vi "Ch_Defaults.vi"(11 "error in":errorcluster) -> (4 "Channels":T1(array[cluster]), 15 "error out":errorcluster)   [LabVIEW 2026]
doc: "128채널 기본 Channel 배열(이름 CH001~CH128, 스케일 0~100 %, 상한 80/하한 20, 저장 ON, 그래프 CH001~CH008)."
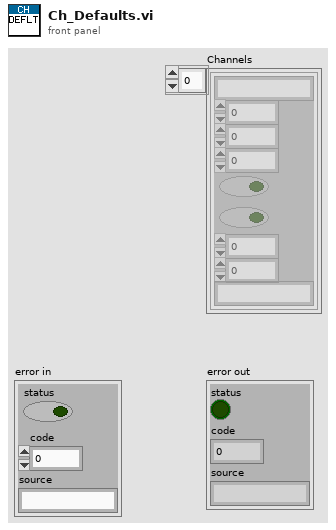
[diagram p1: front panel]
types:
  T1 = cluster{"Name":string, "Value":dbl, "High Limit":dbl, "Low Limit":dbl, "Save":bool, "Graph":bool, "Scale Min":dbl, "Scale Max":dbl, "Unit":string}[]
  T2 = cluster{"Name":string, "Value":dbl, "High Limit":dbl, "Low Limit":dbl, "Save":bool, "Graph":bool, "Scale Min":dbl, "Scale Max":dbl, "Unit":string}
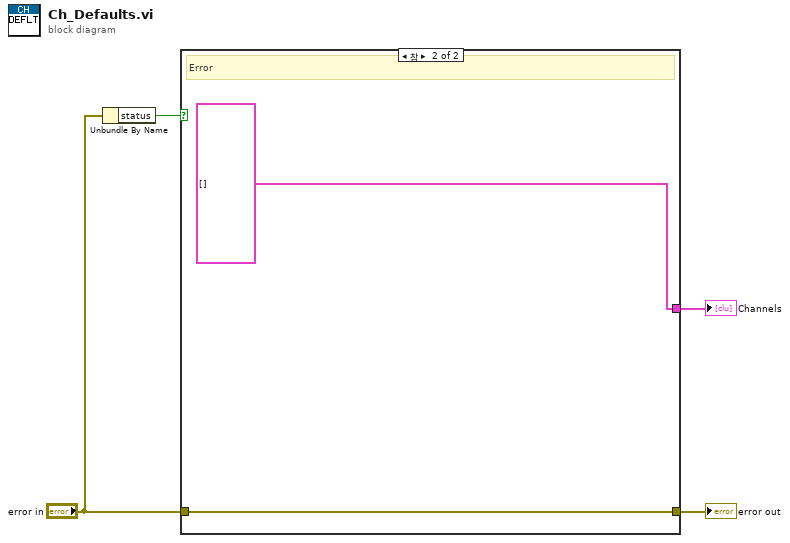
[diagram p0: block diagram]
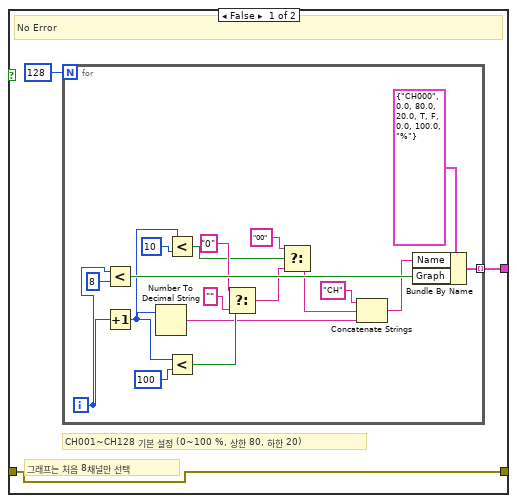
[diagram p2: hidden frame]
diagram:
  n1 = Unbundle By Name("error in") -> ("status"=w2:bool)
  n2 = case shown="참" w2 {
    tunnel: "error in" -> [w5 w26]
    tunnel: [w5 w26] -> w4
    tunnel: [w7 T1 []] -> w3
    frame False {
      # "그래프는 처음 8채널만 선택"
      # "CH001~CH128 기본 설정 (0~100 %, 상한 80, 하한 20)"
      # "No Error"
      n3 = for {
        N: 128 -> [_]
        tunnel: [w25] -> w7 mode=indexing
        i -> [w8]
        n4 = Less?(x=w8, y=8) -> (x < y?=w23:bool)
        n5 = Increment(x=w8) -> (x+1=w9:i32)
        n6 = Number To Decimal String(number=w9) -> (decimal integer string=w10:string)  [unwired: 1 in]
        n7 = Less?(x=w9, y=10) -> (x < y?=w12:bool)
        n8 = Less?(x=w9, y=100) -> (x < y?=w15:bool)
        n9 = Select(t="0", s=w15, f="") -> (s? t:f=w18:string)
        n10 = Select(t="00", s=w12, f=w18) -> (s? t:f=w19:string)
        n11 = Concatenate Strings("CH", w19, w10) -> (w21:string)
        n12 = Bundle By Name(cluster=T2 {"Name"="CH000", "Value"=0.0, "High Limit"=80.0, "Low Limit"=20.0, "Save"=TRUE, "Graph"=FALSE, "Scale Min"=0.0, "Scale Max"=100.0, "Unit"="%"}, "Name"=w21, "Graph"=w23) -> (w25:T2)
      }
    }
    frame True {
      # "Error"
    }
  }
  "Channels" <- w3
  "error out" <- w4
